vi "Create Type Definitions.vi"(8 "error in":errorcluster, 11 "Runner in":refnum<class "Runner.lvclass">) -> (0 "error out":errorcluster, 3 "Runner out":refnum<class "Runner.lvclass">)   [LabVIEW 2026, in "Runner.lvlib" / "Runner.lvclass"]
doc: "Create type definitions (dummy) files from template."
uses:
  Runner.lvclass
  Runner.lvclass/Runner.ctl
  Interfaces/ILogger/ILogger Messages/Log Msg/Log Msg.lvclass/Log Msg.ctl
  <vilib>/ActorFramework/Message Enqueuer/Message Enqueuer.lvclass/Message Enqueuer.ctl
  <vilib>/ActorFramework/Message Enqueuer/Enqueue.vi
  Interfaces/ILogger/ILogger Messages/Log Msg/Log Msg.lvclass
  <vilib>/ActorFramework/Message Priority Queue/Priority Enqueue.vi
  Interfaces/IFile Manager/IFile Manager.lvclass
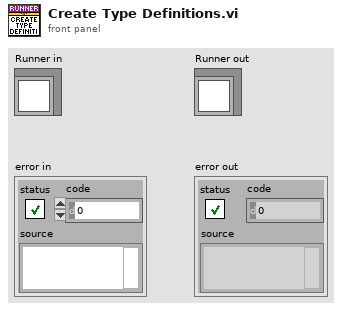
[diagram p1: front panel]
types:
  T1 = typedef "Type Definition--cluster.ctl" = cluster{"name":string, "fields":T2[]}
  T2 = typedef "Parameter--cluster.ctl" = cluster{"name":string, "data_type":string, "container":string, "dimensions":i32, "type_definition":string}
  T3 = typedef "Log Entry--cluster.ctl" = cluster{"Time":timestamp, "Message":string}
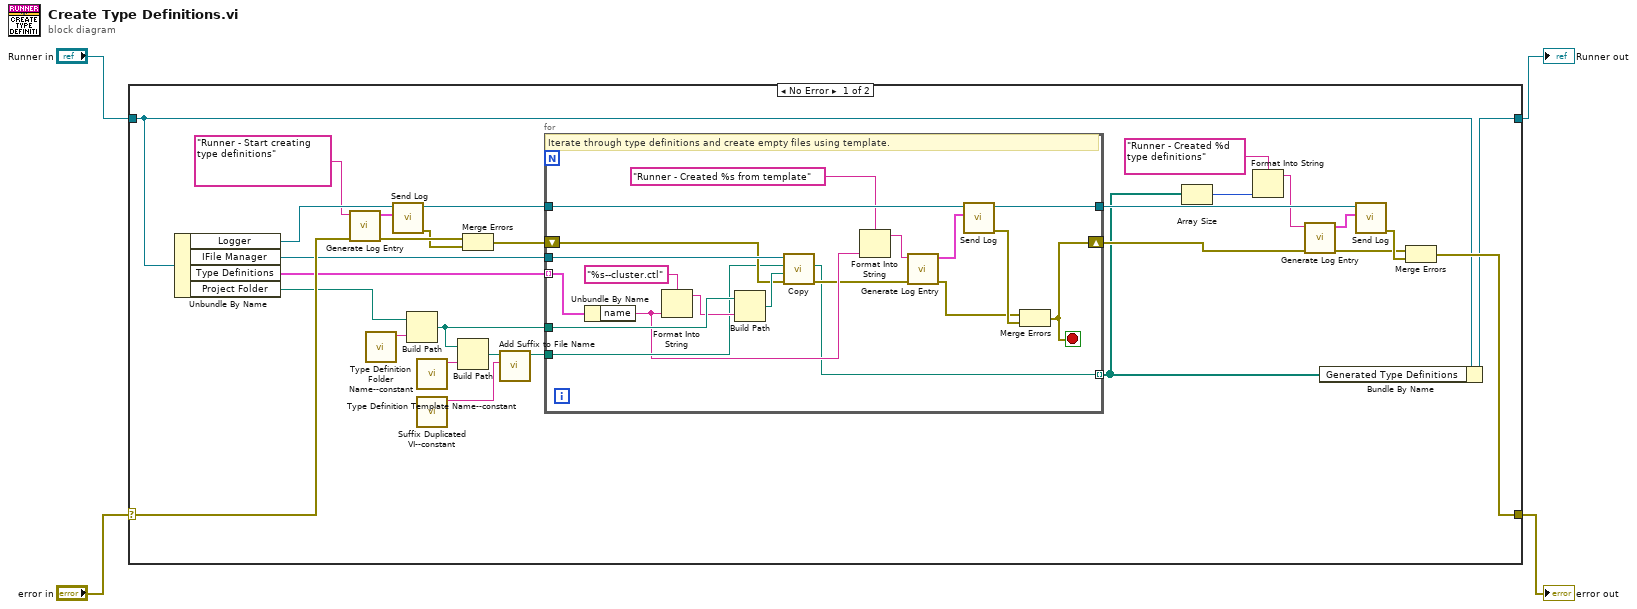
[diagram p0: block diagram]
diagram:
  n1 = case shown="No Error" "error in" {
    selector: "error in" -> [w26 w54]
    tunnel: [w30 w54] -> w2
    tunnel: "Runner in" -> [w25 w53]
    tunnel: [w20 w53] -> w1
    frame No Error {
      n2 = Unbundle By Name(w25) -> ("Logger"=w18:refnum<class "Message Enqueuer.lvclass">, "IFile Manager"=w6:refnum<class "IFile Manager.lvclass">, "Type Definitions"=w24:T1[], "Project Folder"=w19:path)
      n3 = call "Generate Log Entry.vi"("error in"=w26, "Message"="Runner - Start creating type definitions") -> ("error out"=w33:errorcluster, "Log Entry"=w16:T3)  [unwired: 8 in]
      n4 = call "Type Definition Folder Name--constant.vi"() -> ("Type Definition Folder Name"=w23:string)  [unwired: 11 in]
      n5 = call "Send Log.vi"("Log Entry"=w16, "Message Enqueuer"=w18) -> ("error out"=w31:errorcluster, "Message Enqueuer out"=w17:refnum<class "Message Enqueuer.lvclass">)  [unwired: 8 in]
      n6 = Build Path(base path=w19, name or relative path=w23) -> (appended path=w22:path)
      n7 = call "Type Definition Template Name--constant.vi"() -> ("Type Definition Template Name"=w21:string)  [unwired: 11 in]
      n8 = call "Suffix Duplicated VI--constant.vi"() -> ("Suffix Duplicated VI"=w7:string)  [unwired: 11 in]
      n9 = Build Path(base path=w22, name or relative path=w21) -> (appended path=w9:path)
      n10 = Merge Errors(w33, w31) -> (w32:errorcluster)
      n11 = call "Add Suffix to File Name.vi"("Suffix"=w7, "File Path in"=w9) -> ("File Path out"=w8:path)  [unwired: 9 in]
      n12 = for {
        tunnel: w24 -> [w50] mode=indexing
        tunnel: w22 -> [w42]
        shift-right: [w51] -> w28
        shift-left: w32 -> [w39]
        tunnel: w8 -> [w38]
        tunnel: w17 -> [w49]
        tunnel: [w45] -> w13
        tunnel: w6 -> [w44]
        tunnel: [w34] -> w5 mode=indexing
        stop <- w51 stop-if-true
        # "Iterate through type definitions and create empty files using template."
        n13 = Unbundle By Name(w50) -> ("name"=w37:string)
        n14 = Format Into String(format string="%s--cluster.ctl", w37) -> (resulting string=w41:string)  [unwired: 2 in, 1 out]
        n15 = Build Path(base path=w42, name or relative path=w41) -> (appended path=w40:path)
        n16 = call-dynamic "Copy.vi"("error in"=w39, "Target Folder"=w40, "Source File"=w38, "IFile Manager in"=w44) -> ("error out"=w36:errorcluster, "New Path"=w34:path)  [unwired: 5 in, 1 out]
        n17 = Format Into String(format string="Runner - Created %s from template", w37) -> (resulting string=w47:string)  [unwired: 2 in, 1 out]
        n18 = call "Generate Log Entry.vi"("error in"=w36, "Message"=w47) -> ("error out"=w35:errorcluster, "Log Entry"=w46:T3)  [unwired: 8 in]
        n19 = call "Send Log.vi"("Log Entry"=w46, "Message Enqueuer"=w49) -> ("error out"=w52:errorcluster, "Message Enqueuer out"=w45:refnum<class "Message Enqueuer.lvclass">)  [unwired: 8 in]
        n20 = Merge Errors(w35, w52) -> (w51:errorcluster)
      }
      n21 = Array Size(array=w5) -> (size(s)=w11:i32)
      n22 = Format Into String(format string="Runner - Created %d type definitions" ("Message"), w11) -> (resulting string=w10:string)  [unwired: 2 in, 1 out]
      n23 = call "Generate Log Entry.vi"("error in"=w28, "Message"=w10) -> ("error out"=w27:errorcluster, "Log Entry"=w14:T3)  [unwired: 8 in]
      n24 = Bundle By Name(cluster=w25, "Generated Type Definitions"=w5) -> (w20:refnum<class "Runner.lvclass">)
      n25 = call "Send Log.vi"("Log Entry"=w14, "Message Enqueuer"=w13) -> ("error out"=w29:errorcluster)  [unwired: 8 in, 1 out]
      n26 = Merge Errors(w27, w29) -> (w30:errorcluster)
    }
    frame Error {
      # "Pass error"
    }
  }
  "error out" <- w2
  "Runner out" <- w1
